vi "plcm3CloseUnit.vi"(8 "error in (no error)":errorcluster, 11 "handle in":i16=16384) -> (0 "error out":errorcluster, 3 "handle out":i16)   [LabVIEW 2010]
doc: "This closes the device and should be called before exiting an application."
uses:
  plcm3.dll
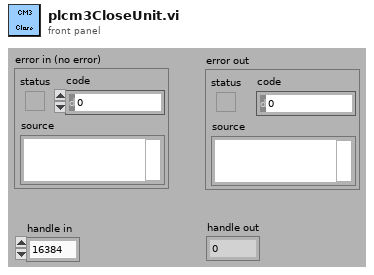
[diagram p1: front panel]
types:
  T1 = cluster{"status":bool, "code":u32, "source":string}
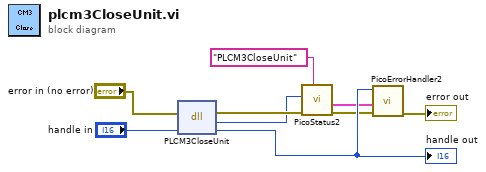
[diagram p0: block diagram]
diagram:
  n1 = dll-call lib="plcm3.dll" fn="PLCM3CloseUnit"(error in="error in (no error)", "handle"="handle in") -> (error out=w4:errorcluster, "Status"=w1:u32, "handle"=w8:i16)  [unwired: 2 in, 1 out]
  "handle out" <- w8
  n2 = call "PicoStatus2.vi"("PICO source"="PLCM3CloseUnit" ("source"), "Error in"=w4, "PICO STATUS"=w1) -> ("error out"=w5:errorcluster, "PICO_STATUS out"=w2:T1)  [unwired: 5 in]
  n3 = call "PicoErrorHandler2.vi"("error in (no error)"=w5, "PICO_STATUS in"=w2, "handle In"=w8) -> ("error out"=→"error out":errorcluster)  [unwired: 8 in]
